vi "work1_takeorder_and_cook.vi"() -> ()   [LabVIEW 2026]
panel:
  in  "stop":bool
  out "Clients Served":i16
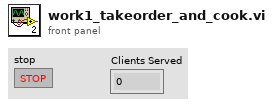
[diagram p1: front panel]
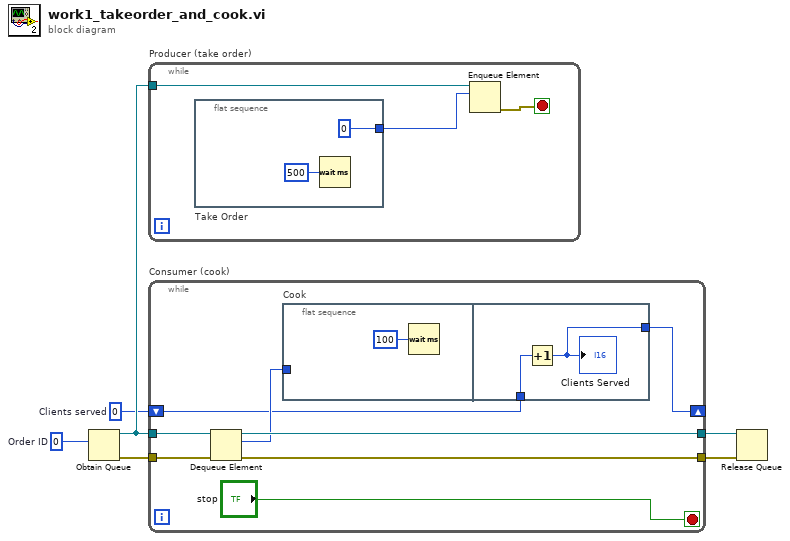
[diagram p0: block diagram]
diagram:
  w1 = i16 0  # Clients served
  w2 = 0  # Order ID
  n1 = Obtain Queue(element data type=w2) -> (queue out=w5:refnum<queue>, error out=w4:errorcluster)  [unwired: 4 in, 1 out]
  n2 = while "Producer (take order)" {
    tunnel: w5 -> [w9]
    stop <- w8 stop-if-true
    n3 = flat-sequence "Take Order" {
      tunnel: [0] -> w7
      frame #0 {
        n4 = Wait (ms)(milliseconds to wait=u32 500) -> ()  [unwired: 1 out]
      }
    }
    n5 = Enqueue Element(queue=w9, element=w7) -> (error out=w8:errorcluster)  [unwired: 2 in, 2 out]
  }
  n6 = while "Consumer (cook)" {
    tunnel: w5 -> [w19]
    tunnel: [w18] -> w6
    tunnel: w4 -> [w17]
    tunnel: [w16] -> w3
    shift-right: [w12] -> _
    shift-left: w1 -> [w14]
    stop <- "stop" stop-if-true
    n7 = Dequeue Element(queue=w19, error in (no error)=w17) -> (queue out=w18:refnum<queue>, element=w15:i32, error out=w16:errorcluster)  [unwired: 1 in, 1 out]
    n8 = flat-sequence "Cook" {
      tunnel: w15 -> [_]
      tunnel: w14 -> [w22]
      tunnel: [w21] -> w12
      frame #0 {
        n9 = Wait (ms)(milliseconds to wait=u32 100) -> ()  [unwired: 1 out]
      }
      frame #1 {
        n10 = Increment(x=w22) -> (x+1=w21:i16)
        "Clients Served" <- w21
      }
    }
  }
  n11 = Release Queue(queue=w6, error in (no error)=w3) -> ()  [unwired: 1 in, 3 out]
